vi "FuncVI-smatch.vi"(5 "InstanceRef":T2, 9 "arg list":T1[](array[typedef]) {"num" format="%.2f"}) -> (0 "error out":bool, 3 "result":T1 {"num" format="%.2f"})   [LabVIEW 2021]
doc: "::: CalcExpress Toolkit :::\nCopyright (c) 2000-2026 Konstantin Shifershteyn. All rights reserved."
uses:
  cetypes.llb/CalcExpress Function Argument Info.ctl
  cetypes.llb/CalcExpress Instance RefNum.ctl
panel:
  in  "max arg num":i32=3
  in  "min arg num":i32=2
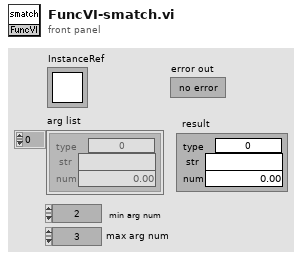
[diagram p1: front panel]
types:
  T1 = typedef "CalcExpress Function Argument Info.ctl" = cluster{"type":u32, "str":string, "num":dbl}
  T2 = typedef "CalcExpress Instance RefNum.ctl" = refnum<k1>
  T3 = enum32{"String", "DBL Number", "identifier", "1D Array of DBL", "2D Array of DBL", "CDB Number", "1D Array of CDB", "2D Array of CDB", "1D Array of String", "2D Array of String", "Unknown data type"}
  T4 = cluster{"index":i32, "any type":i32, "default num":dbl, "default str":string}
  T5 = cluster{"index":i32, "data type":enum32{"String", "DBL Number", "identifier", "1D Array of DBL", "2D Array of DBL", "CDB Number", "1D Array of CDB", "2D Array of CDB", "1D Array of String", "2D Array of String", "Unknown data type"}, "default num":dbl, "default str":string}[]
  T6 = cluster{"index":i32, "data type":u32, "default num":dbl, "default str":string}[]
  T7 = cluster{"data type":enum32{"String", "DBL Number", "identifier", "1D Array of DBL", "2D Array of DBL", "CDB Number", "1D Array of CDB", "2D Array of CDB", "1D Array of String", "2D Array of String", "Unknown data type"}, "data string":string, "num":dbl}
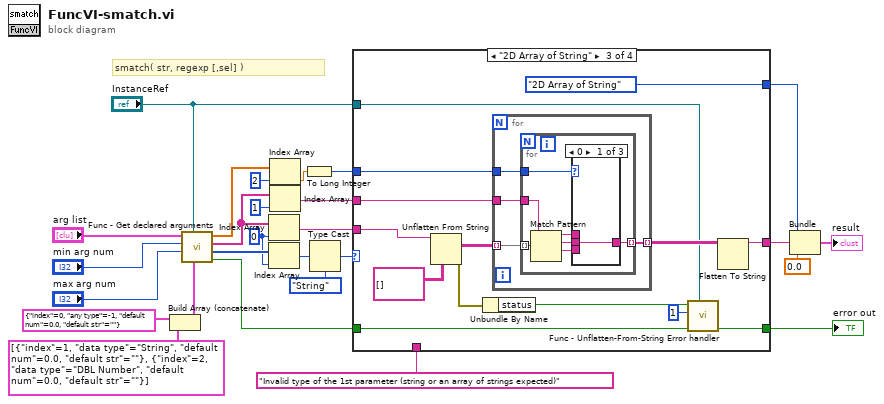
[diagram p0: block diagram]
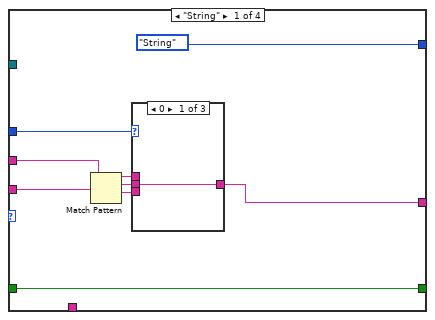
[diagram p2: hidden frame]
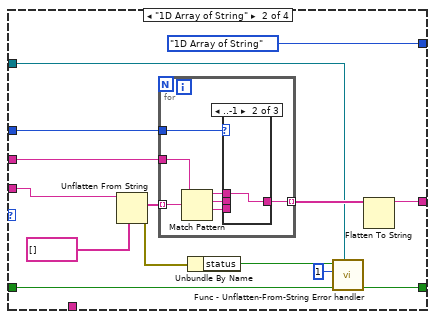
[diagram p5: hidden frame]
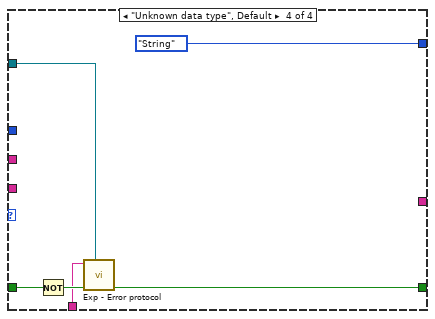
[diagram p10: hidden frame]
diagram:
  w14 = 0
  # "smatch( str, regexp [,sel] )"
  n1 = Build Array (concatenate)(T4 {"index"=0, "any type"=-1, "default num"=0.0, "default str"=""} ("arg descriptor"), T5 [{"index"=1, "data type"=enum."String", "default num"=0.0, "default str"=""}, {"index"=2, "data type"=enum."DBL Number", "default num"=0.0, "default str"=""}] ("args descriptors")) -> (w20:T6)
  n2 = call "Func - Get declared arguments.vi"("arg descriptors"=w20, "InstanceRef"="InstanceRef", "max arg num"="max arg num", "min arg num"="min arg num", "arg list"="arg list") -> ("error out"=w13:bool, "type list"=w15:u32[], "str list"=w9:string[], "num list"=w8:dbl[])  [unwired: 3 in]
  n3 = Index Array(array=w9, index=w14) -> (element=w16:string)
  n4 = Index Array(array=w15, index=w14) -> (element=w17:u32)
  n5 = Index Array(array=w8, index=2) -> (element=w24:dbl)
  n6 = Index Array(array=w9, index=1) -> (element=w25:string)
  n7 = To Long Integer(number=w24) -> (32bit integer=w7:i32)
  n8 = Type Cast(type=T3."String" ("data type"), x=w17) -> (*(type *) &x=w18:T3)
  n9 = case shown="\"2D Array of String\"" w18 {
    tunnel: w16 -> [w34 w53 w76 _]
    tunnel: [w28 w49 w72 _] -> w6
    tunnel: w25 -> [w33 w47 w70 _]
    tunnel: w7 -> [w32 w51 w74 _]
    tunnel: w13 -> [w36 w43 w68 w97]
    tunnel: [w36 w42 w69 w95] -> w12
    tunnel: "Invalid type of the 1st parameter (string or an array of strings expected)" ("ErrStr") -> [_ _ _ w94]
    tunnel: "InstanceRef" -> [_ w46 w65 w93]
    tunnel: [T3."String" ("data type") T3."1D Array of String" ("data type") T3."2D Array of String" ("data type") T3."String" ("data type")] -> w4
    frame "String" {
      n10 = Match Pattern(string=w34, regular expression=w33) -> (before substring=w29:string, match substring=w31:string, after substring=w30:string)  [unwired: 1 in, 1 out]
      n11 = case shown="0" w32 {
        tunnel: w29 -> [_ w38 _]
        tunnel: w31 -> [w37 _ _]
        tunnel: w30 -> [_ _ w39]
        tunnel: [w37 w38 w39] -> w28
        frame 0 {
        }
        frame ..-1 {
        }
        frame 1.. {
        }
      }
    }
    frame "1D Array of String" {
      n12 = Unflatten From String(type=string[] [], binary string=w53) -> (value=w52:string[], error out=w41:errorcluster)  [unwired: 3 in, 1 out]
      n13 = for {
        tunnel: w52 -> [w60] mode=indexing
        tunnel: w51 -> [w59]
        tunnel: [w58] -> w50 mode=indexing
        tunnel: w47 -> [w54]
        n14 = Match Pattern(string=w60, regular expression=w54) -> (before substring=w55:string, match substring=w57:string, after substring=w56:string)  [unwired: 1 in, 1 out]
        n15 = case shown="..-1" w59 {
          tunnel: w55 -> [_ w62 _]
          tunnel: w57 -> [w61 _ _]
          tunnel: w56 -> [_ _ w63]
          tunnel: [w61 w62 w63] -> w58
          frame 0 {
          }
          frame ..-1 {
          }
          frame 1.. {
          }
        }
      }
      n16 = Unbundle By Name(w41) -> ("status"=w45:bool)
      n17 = call "Func - Unflatten-From-String Error handler.vi"("InstanceRef"=w46, "error in"=w43, "argument number"=1, "Unflatten Error status"=w45) -> ("error out"=w42:bool)  [unwired: 5 in]
      n18 = Flatten To String(anything=w50) -> (data string=w49:string)  [unwired: 3 in, 2 out]
    }
    frame "2D Array of String" {
      n19 = Unflatten From String(type=string[][] [], binary string=w76) -> (value=w75:string[][], error out=w64:errorcluster)  [unwired: 3 in, 1 out]
      n20 = Unbundle By Name(w64) -> ("status"=w67:bool)
      n21 = for {
        tunnel: w75 -> [w81] mode=indexing
        tunnel: w74 -> [w80]
        tunnel: [w79] -> w73 mode=indexing
        tunnel: w70 -> [w78]
        n22 = for {
          tunnel: w81 -> [w85] mode=indexing
          tunnel: w80 -> [w84]
          tunnel: [w83] -> w79 mode=indexing
          tunnel: w78 -> [w82]
          n23 = Match Pattern(string=w85, regular expression=w82) -> (before substring=w86:string, match substring=w88:string, after substring=w87:string)  [unwired: 1 in, 1 out]
          n24 = case shown="0" w84 {
            tunnel: w86 -> [_ w90 _]
            tunnel: w88 -> [w89 _ _]
            tunnel: w87 -> [_ _ w91]
            tunnel: [w89 w90 w91] -> w83
            frame 0 {
            }
            frame ..-1 {
            }
            frame 1.. {
            }
          }
        }
      }
      n25 = call "Func - Unflatten-From-String Error handler.vi"("InstanceRef"=w65, "error in"=w68, "argument number"=1, "Unflatten Error status"=w67) -> ("error out"=w69:bool)  [unwired: 5 in]
      n26 = Flatten To String(anything=w73) -> (data string=w72:string)  [unwired: 3 in, 2 out]
    }
    frame "Unknown data type", Default {
      n27 = Not(x=w97) -> (.not. x?=w96:bool)
      n28 = call "Exp - Error protocol.vi"("InstanceRef"=w93, "error in"=w96, "error message in"=w94) -> ("error out"=w95:bool)  [unwired: 5 in, 1 out]
    }
  }
  "error out" <- w12
  n29 = Bundle("data type"=w4, "data string"=w6, "num"=0.0) -> (→"result":T7)  [unwired: 1 in]
